vi "Read value (Boolean).vi"(8 "error in (no error)":errorcluster, 9 "default value":bool, 11 "JSON Boolean in":refnum<class "JSON Value.lvclass">) -> (0 "error out":errorcluster, 1 "defaulted?":bool, 2 "value":bool)   [LabVIEW 2017, in "JSON Value.lvclass"]
doc: "Returns the value of a JSON Boolean"
uses:
  JSON Value.lvclass
  JSON Value.lvclass/JSON Value.ctl
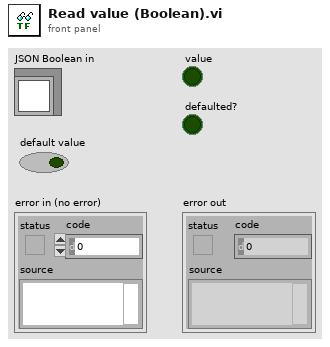
[diagram p1: front panel]
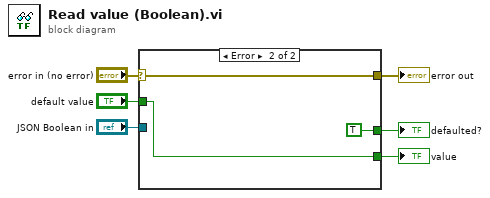
[diagram p0: block diagram]
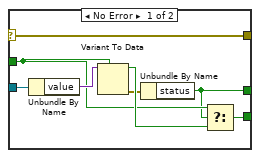
[diagram p2: hidden frame]
diagram:
  n1 = case shown="Error" "error in (no error)" {
    selector: "error in (no error)" -> [w14 w17]
    tunnel: [w14 w17] -> w5
    tunnel: "JSON Boolean in" -> [w13 _]
    tunnel: [w9 w16] -> w3
    tunnel: "default value" -> [w10 w16]
    tunnel: [w7 TRUE ("status")] -> w1
    frame No Error {
      n2 = Unbundle By Name(w13) -> ("value"=w12:variant)
      n3 = Variant To Data(type=w10, Variant=w12) -> (data=w11:bool, error out=w8:errorcluster)  [unwired: 1 in]
      n4 = Unbundle By Name(w8) -> ("status"=w7:bool)
      n5 = Select(t=w10, s=w7, f=w11) -> (s? t:f=w9:bool)
    }
    frame Error {
    }
  }
  "error out" <- w5
  "value" <- w3
  "defaulted?" <- w1
